vi "TIME.vi"(1 "Numeric 2":i32, 2 "y":i32) -> (0 "Numeric":dbl)   [LabVIEW 2026]
panel:
  out "Numeric 5":dbl
  out "Numeric 4":i32
  out "Numeric 3":dbl
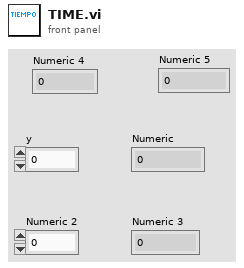
[diagram p1: front panel]
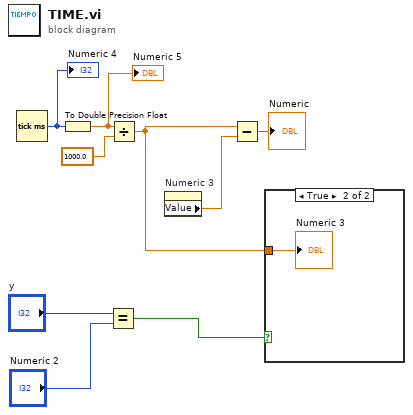
[diagram p0: block diagram]
diagram:
  n1 = Tick Count (ms)() -> (millisecond timer value=w1:u32)
  "Numeric 4" <- w1
  n2 = To Double Precision Float(number=w1) -> (double precision float=w2:dbl)
  "Numeric 5" <- w2
  n3 = Equal?(x="y", y="Numeric 2") -> (x = y?=w9:bool)
  n4 = Divide(x=w2, y=1000.0) -> (x/y=w5:dbl)
  n5 = property on="Numeric 3" class="DigNum (strict)"() -> ("Value"=w6:dbl)  [unwired: 2 in, 2 out]
  n6 = Subtract(x=w5, y=w6) -> (x-y=→"Numeric":dbl)
  n7 = case shown="True" w9 {
    tunnel: w5 -> [_ w10]
    frame False {
    }
    frame True {
      "Numeric 3" <- w10
    }
  }
